vi "ROI coord bundler.vi"(0 "Experiment folder path":path, 5 "error in (no error)":errorcluster) -> (6 "Number of POIs":i32, 7 "Zoom":dbl[](array[numeric]), 10 "variable X Miniscan Pixels":i32[](array[numeric]), 11 "ROI Attributes (broken down to miniscans)":T1[](array[typedef]) {"Apparent Frame Size" format="%#_6f"; "Original FOV (um)" format="%#_6f"; "Pixels per miniscan" format="%#_6f"; "Dwell Time per pixel" format="%#_6f"; "Resolution" format="%#_6f"; "ROI group ID" format="%#_6f"; "Laser Power (%)" format="%#_6f"; "Zoom" format="%#_6f"; "Frame Size" format="%#_6f"; "Number of lines" format="%#_6f"; "Composite ID" format="%#_6f"; "Angle (deg)" format="%#_6f"; "ROI Time (ns)" format="%#_6f"; "ROI ID" format="%#_6f"; "Pixels in ROI" format="%#_6f"; "ROI index" format="%#_6f"; "Z stop" format="%#_6f"; "Y stop" format="%#_6f"; "X stop" format="%#_6f"; "Z start" format="%#_6f"; "X start" format="%#_6f"; "Y start" format="%#_6f"}, 12 "Number of pixels in single miniscan":i32, 13 "Laser(V)":dbl[](array[numeric]), 14 "ROI Coordinates (broken down to miniscans)":T2, 15 "Total number of miniscans":i32, 17 "Total Pixels":i32, 18 "ROI Attributes":T1[](array[typedef]) {"Apparent Frame Size" format="%#_6f"; "Original FOV (um)" format="%#_6f"; "Pixels per miniscan" format="%#_6f"; "Dwell Time per pixel" format="%#_6f"; "Resolution" format="%#_6f"; "ROI group ID" format="%#_6f"; "Laser Power (%)" format="%#_6f"; "Zoom" format="%#_6f"; "Frame Size" format="%#_6f"; "Number of lines" format="%#_6f"; "Composite ID" format="%#_6f"; "Angle (deg)" format="%#_6f"; "ROI Time (ns)" format="%#_6f"; "ROI ID" format="%#_6f"; "Pixels in ROI" format="%#_6f"; "ROI index" format="%#_6f"; "Z stop" format="%#_6f"; "Y stop" format="%#_6f"; "X stop" format="%#_6f"; "Z start" format="%#_6f"; "X start" format="%#_6f"; "Y start" format="%#_6f"}, 19 "error out":errorcluster)   [LabVIEW 2020]
uses:
  User Interface/Visualisation/Functional Imaging Viewer/Typedefs/ROI parameters data type.ctl
  Typedefs/ROI XY coordinates cluster.ctl
panel:
  # "PRE-ALLOCATED CLONE RE-ENTRANT"
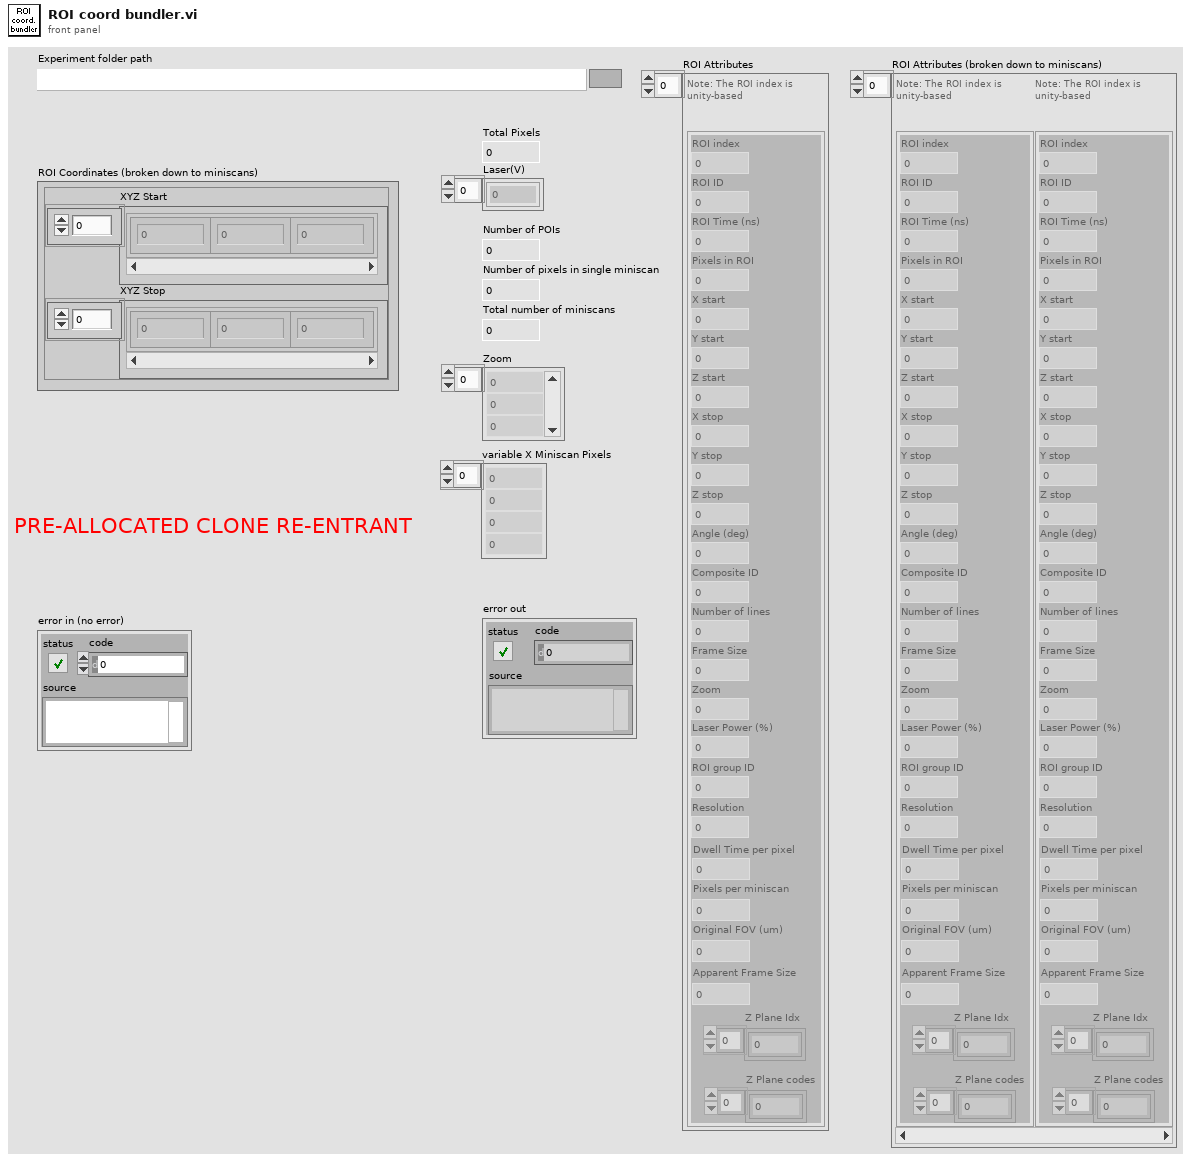
[diagram p1: front panel]
types:
  T1 = typedef "ROI parameters data type.ctl" = cluster{"ROI index":dbl, "ROI ID":dbl, "ROI Time (ns)":dbl, "Pixels in ROI":dbl, "X start":dbl, "Y start":dbl, "Z start":dbl, "X stop":dbl, "Y stop":dbl, "Z stop":dbl, "Angle (deg)":dbl, "Composite ID":dbl, "Number of lines":dbl, "Frame Size":dbl, "Zoom":dbl, "Laser Power (%)":dbl, "ROI group ID":dbl, "Resolution":dbl, "Dwell Time per pixel":dbl, "Pixels per miniscan":dbl, "Original FOV (um)":dbl, "Apparent Frame Size":dbl, "Z Plane Idx":i32[], "Z Plane codes":i32[]}
  T2 = typedef "ROI XY coordinates cluster.ctl" = cluster{"XYZ Start":cluster{"X":sgl, "Y":sgl, "Z":sgl}[], "XYZ Stop":cluster{"X":sgl, "Y":sgl, "Z":sgl}[]}
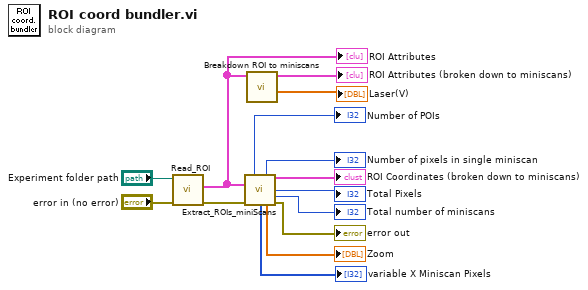
[diagram p0: block diagram]
diagram:
  n1 = call "Read_ROI.vi"("error in"="error in (no error)", "Experiment folder path"="Experiment folder path") -> ("error out"=w12:errorcluster, "ROI setup"=w5:T1[])  [unwired: 8 in]
  "ROI Attributes" <- w5
  n2 = call "Extract_ROIs_miniScans.vi"("ROI Attributes"=w5, "error in (no error)"=w12) -> ("number of POI"=→"Number of POIs":i32, "Number of pixels in single X miniscan"=→"Number of pixels in single miniscan":i32, "ROI Coordinates (broken down to miniscans)"=→"ROI Coordinates (broken down to miniscans)":T2, "Total Pixels"=→"Total Pixels":i32, "Total number of miniscans"=→"Total number of miniscans":i32, "variable X Miniscan Pixels"=→"variable X Miniscan Pixels":i32[], "Zoom"=→"Zoom":dbl[], "error out"=→"error out":errorcluster)  [unwired: 4 in, 2 out]
  n3 = call "Breakdown ROI to miniscans.vi"("ROI Attributes"=w5) -> ("Laser(V)"=→"Laser(V)":dbl[], "ROI Attributes (broken down to miniscans)"=→"ROI Attributes (broken down to miniscans)":T1[])  [unwired: 9 in]
